vi "Parameter.vi"(8 "error in (no error)":errorcluster, 11 "Node Ptr":T2 format="%.0x") -> (0 "error out":errorcluster)   [LabVIEW 2020, in "AIM ARINC 429 System Explorer.lvlib" / "Implementation.lvlib"]
uses:
  Implementation.lvlib
  <vilib>/NI VeriStand/Custom Device API/Custom Device API.lvlib
  Scripting/AIM/AIM ARINC 429 Scripting.lvlib
  <vilib>/NI VeriStand/Custom Device API/Custom Device Item Ref.ctl
  <vilib>/NI/NI VeriStand Encoding and Decoding/Encoding.ctl
  <vilib>/NI/NI VeriStand Encoding and Decoding/Encoding and Decoding.lvlib
panel:
  out "Unit":string
  out "Scale Offset":dbl
  out "Scale Factor":dbl=1.0
  out "Signed?":bool=TRUE
  out "Number of Bits":i32=10
  out "Start Bit":i32=18
  out "Default Value (Scaled)":dbl
  out "Encoding Type":T1
  in  "SHDocVw.IWebBrowser":refnum<k7>(container)
  in  "General Header":cluster{"Section Name":string}={"Section Name"="ARINC 429 - Parameter"}
  in  "Description":string
  out "Name":string
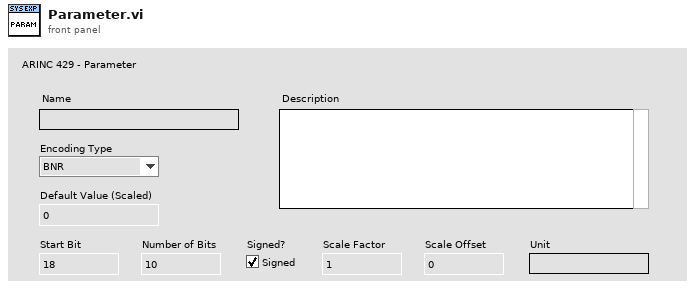
[diagram p1: front panel]
types:
  T1 = typedef "Encoding and Decoding.lvlib/Encoding.ctl" = enum16{"BNR", "BCD", "Discrete"}
  T2 = typedef "Custom Device API.lvlib/Custom Device Item Ref.ctl" = u64
  T3 = typedef "Custom Device API.lvlib/Custom Device Item Info.ctl" = cluster{"Name":string, "Is Channel":bool, "GUID":string, "Is Waveform":bool}
  T4 = typedef "Parameter Definition.ctl" = cluster{"start index":i32, "size":i32, "encoding":T1, "signed":bool, "scale multiplier":dbl, "scale offset":dbl, "default value":dbl}
  T5 = typedef "Custom Device API.lvlib/Custom Device Commands.ctl" = enum16{"Default", "Item renamed", "Shutdown", "Dynamic button pressed"}
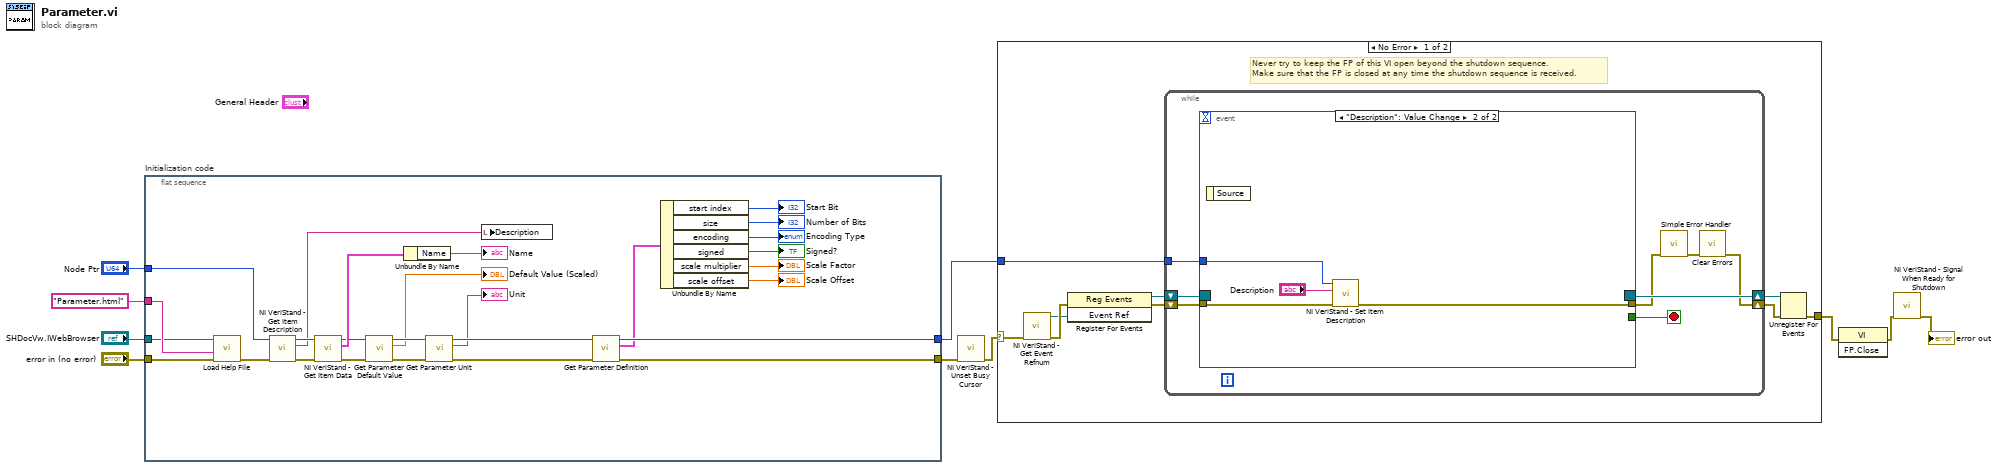
[diagram p0: block diagram]
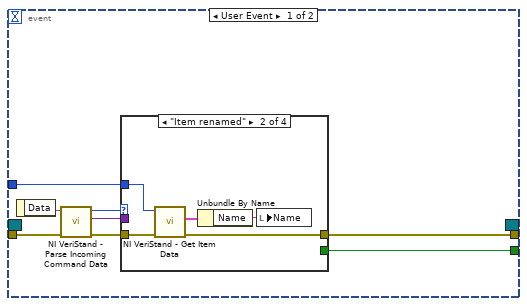
[diagram p2: hidden frame]
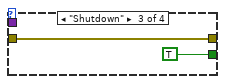
[diagram p4: hidden frame]
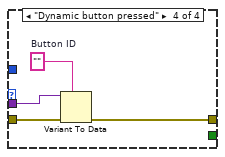
[diagram p5: hidden frame]
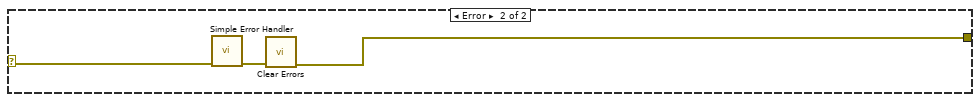
[diagram p6: hidden frame]
diagram:
  n1 = flat-sequence "Initialization code" {
    tunnel: "error in (no error)" -> [w32]
    tunnel: "Node Ptr" -> [w34]
    tunnel: [w27] -> w6
    tunnel: [w26] -> w3
    tunnel: "SHDocVw.IWebBrowser" -> [w29]
    tunnel: "Parameter.html" ("CD_CHM_Section") -> [w30]
    frame #0 {
      n2 = call "Load Help File.vi"("error in (no error)"=w32, "HTML File to Load"=w30, "Browser"=w29) -> ("error out"=w31:errorcluster)  [unwired: 8 in]
      n3 = call <vilib>:"NI VeriStand - Get Item Description.vi"("error in (no error)"=w31, "Item Ref in"=w34) -> ("error out"=w36:errorcluster, "Description"=w33:string, "Item Ref out"=w37:T2)  [unwired: 7 out]
      n4 = call <vilib>:"NI VeriStand - Get Item Data.vi"("error in (no error)"=w36, "Item Ref in"=w37) -> ("error out"=w14:errorcluster, "Item Info"=w35:T3, "Item Ref out"=w15:T2)  [unwired: 7 out]
      n5 = call "Get Parameter Default Value.vi"("error in"=w14, "parameter ref"=w15) -> ("error out"=w13:errorcluster, "Default Value (Scaled)"=→"Default Value (Scaled)":dbl, "parameter ref out"=w12:T2)  [unwired: 7 in]
      n6 = Unbundle By Name(w35) -> ("Name"=→"Name":string)
      n7 = call "Get Parameter Unit.vi"("error in"=w13, "parameter ref"=w12) -> ("error out"=w18:errorcluster, "unit"=→"Unit":string, "parameter ref out"=w17:T2)  [unwired: 7 in]
      n8 = local write "Description"(w33) -> ()
      n9 = call "Get Parameter Definition.vi"("error in"=w18, "parameter ref"=w17) -> ("error out"=w27:errorcluster, "parameter definition"=w25:T4, "parameter ref out"=w26:T2)  [unwired: 7 in]
      n10 = Unbundle By Name(w25) -> ("start index"=→"Start Bit":i32, "size"=→"Number of Bits":i32, "encoding"=→"Encoding Type":T1, "signed"=→"Signed?":bool, "scale multiplier"=→"Scale Factor":dbl, "scale offset"=→"Scale Offset":dbl)
    }
  }
  n11 = call <vilib>:"NI VeriStand - Unset Busy Cursor.vi"("error in (no error)"=w6) -> ("error out"=w5:errorcluster)  [unwired: 10 out]
  n12 = case shown="No Error" w5 {
    selector: w5 -> [w38 w81]
    tunnel: [w43 w79] -> w10
    tunnel: w3 -> [w39 _]
    frame No Error {
      # "Never try to keep the FP of this VI open beyond the shutdown sequence.\nMake sure that the FP is closed at any time the shutdown sequence is received."
      n13 = call <vilib>:"NI VeriStand - Get Event Refnum.vi"("error in (no error)"=w38) -> ("error out"=w46:errorcluster, "Event Ref"=w42:refnum<user-event>)  [unwired: 9 out]
      n14 = register-events(error in=w46, w42) -> (reference out=w40:refnum<event-registration>, error out=w41:errorcluster)  [unwired: 1 in]
      n15 = while {
        tunnel: w39 -> [w50]
        shift-right: [w47] -> w44
        shift-left: w41 -> [w53]
        shift-right: [w54] -> w45
        shift-left: w40 -> [w52]
        stop <- w51 stop-if-true
        n16 = event shown="[1] \"Description\": Value Change" {
          selector: w52 -> [_ _]
          dyn-events: [_ _] -> w54
          timeout: _ -> [_ _]
          tunnel: w53 -> [w62 w77]
          tunnel: [w58 _] -> w51
          tunnel: [w57 w76] -> w49
          tunnel: w50 -> [w56 w78]
          event User Event {
            n17 = event-data() -> ("Data"=w61:string)  [unwired: 1 out]
            n18 = call <vilib>:"NI VeriStand - Parse Incoming Command Data.vi"("error in (no error)"=w62, "Incoming data"=w61) -> ("error out"=w60:errorcluster, "Outgoing data"=w55:variant, "Action"=w59:T5)  [unwired: 7 out]
            n19 = case shown="\"Item renamed\"" w59 {
              tunnel: w60 -> [w63 w68 w69 w74]
              tunnel: [_ _ TRUE _] -> w58
              tunnel: [w63 w65 w69 w71] -> w57
              tunnel: w56 -> [_ w67 _ _]
              tunnel: w55 -> [_ _ _ w73]
              frame "Default", Default {
              }
              frame "Item renamed" {
                n20 = call <vilib>:"NI VeriStand - Get Item Data.vi"("error in (no error)"=w68, "Item Ref in"=w67) -> ("error out"=w65:errorcluster, "Item Info"=w66:T3)  [unwired: 8 out]
                n21 = Unbundle By Name(w66) -> ("Name"=w64:string)
                n22 = local write "Name"(w64) -> ()
              }
              frame "Shutdown" {
              }
              frame "Dynamic button pressed" {
                w72 = ""  # Button ID
                n23 = Variant To Data(error in=w74, type=w72, Variant=w73) -> (error out=w71:errorcluster)  [unwired: 1 out]
              }
            }
          }
          event "Description": Value Change {
            n24 = event-data() -> ()  [unwired: 2 out]
            n25 = call <vilib>:"NI VeriStand - Set Item Description.vi"("error in (no error)"=w77, "Description"="Description", "Item Ref in"=w78) -> ("error out"=w76:errorcluster)  [unwired: 8 out]
          }
        }
        n26 = call <vilib>:"Simple Error Handler.vi"("error in (no error)"=w49) -> ("error out"=w48:errorcluster)  [unwired: 1 in, 7 out]
        n27 = call <vilib>:"Clear Errors.vi"("error in (no error)"=w48) -> ("error out"=w47:errorcluster)  [unwired: 1 in, 5 out]
      }
      n28 = Unregister For Events(event registration refnum=w45, error in=w44) -> (error out=w43:errorcluster)
    }
    frame Error {
      n29 = call <vilib>:"Simple Error Handler.vi"("error in (no error)"=w81) -> ("error out"=w80:errorcluster)  [unwired: 1 in, 7 out]
      n30 = call <vilib>:"Clear Errors.vi"("error in (no error)"=w80) -> ("error out"=w79:errorcluster)  [unwired: 1 in, 5 out]
    }
  }
  n31 = invoke class="VI" method="FP.Close"(error in=w10) -> (error out=w9:errorcluster)  [unwired: 2 in, 2 out]
  n32 = call <vilib>:"NI VeriStand - Signal When Ready for Shutdown.vi"("error in (no error)"=w9) -> ("error out"=→"error out":errorcluster)  [unwired: 10 out]
